vi "getSerializedData.vi"(0 "reference":refnum<class "SegmentedLineEdge.lvclass">, 5 "error in (no error)":errorcluster) -> (14 "reference out":refnum<class "SegmentedLineEdge.lvclass">, 15 "startNode":refnum<class "AbstractNode.lvclass">, 16 "endNode":refnum<class "AbstractNode.lvclass">, 17 "xmlOut":string, 19 "error out":errorcluster)   [LabVIEW 2020, in "SegmentedLineEdge.lvclass"]
doc: "getSerializedData"
uses:
  <resource>/Framework/Providers/Open_GDS/UML/SegmentedLineEdge_class/SegmentedLineEdge.lvclass
  C:/Program Files (x86)/National Instruments/LabVIEW 2020/resource/Framework/Providers/Open_GDS/UML/AbstractEdge_class/AbstractEdge.lvclass
  <resource>/Framework/Providers/Open_GDS/UML/AbstractNode_class/AbstractNode.lvclass
  <resource>/Framework/Providers/Open_GDS/UML/General/Point/Point Point2D.ctl
  <resource>/Framework/Providers/Open_GDS/UML/ArrowHead_class/ArrowHead.lvclass
  <resource>/Framework/Providers/Open_GDS/UML/LineStyle_class/LineStyle.lvclass
  <resource>/Framework/Providers/Open_GDS/UML/AbstractEdge_class/AbstractEdge.lvclass
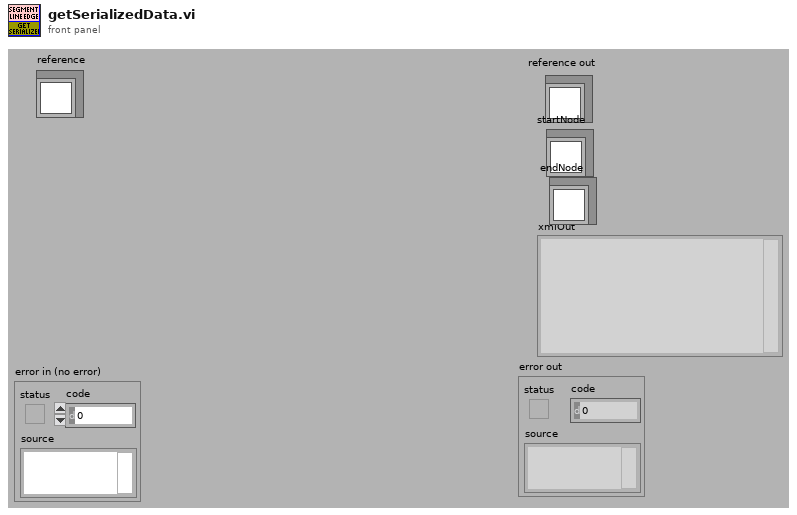
[diagram p1: front panel]
types:
  T1 = typedef "Point Point2D.ctl" = cluster{"x":dbl, "y":dbl}
  T2 = cluster{"Base class":cluster{"Base class":cluster{"start":refnum<k1>, "end":refnum<k1>}}, "lineStyle":refnum<k1>, "startArrowHead":refnum<k1>, "endArrowHead":refnum<k1>, "startLabel":string, "midLabel":string, "endLabel":string, "MidLabelOffset":T1, "SplitWire":bool}
  T3 = typedef "SegmentedLineEdge.lvclass/ObjectAttributes.ctl" = cluster{"lineStyle":refnum<class "LineStyle.lvclass">, "startArrowHead":refnum<class "ArrowHead.lvclass">, "endArrowHead":refnum<class "ArrowHead.lvclass">, "startLabel":string, "midLabel":string, "endLabel":string, "MidLabelOffset":T1, "SplitWire":bool}
  T4 = typedef "AbstractEdge.lvclass/ObjectAttributes.ctl" = cluster{"start":refnum<class "AbstractNode.lvclass">, "end":refnum<class "AbstractNode.lvclass">}
  T5 = cluster{"Base class":cluster{"Base class":cluster{"Base class":cluster{"start":refnum<k1>, "end":refnum<k1>}}, "lineStyle":refnum<k1>, "startArrowHead":refnum<k1>, "endArrowHead":refnum<k1>, "startLabel":string, "midLabel":string, "endLabel":string, "MidLabelOffset":T1, "SplitWire":bool}, "Type(String)":string, "Object name":string, "Object name":string}
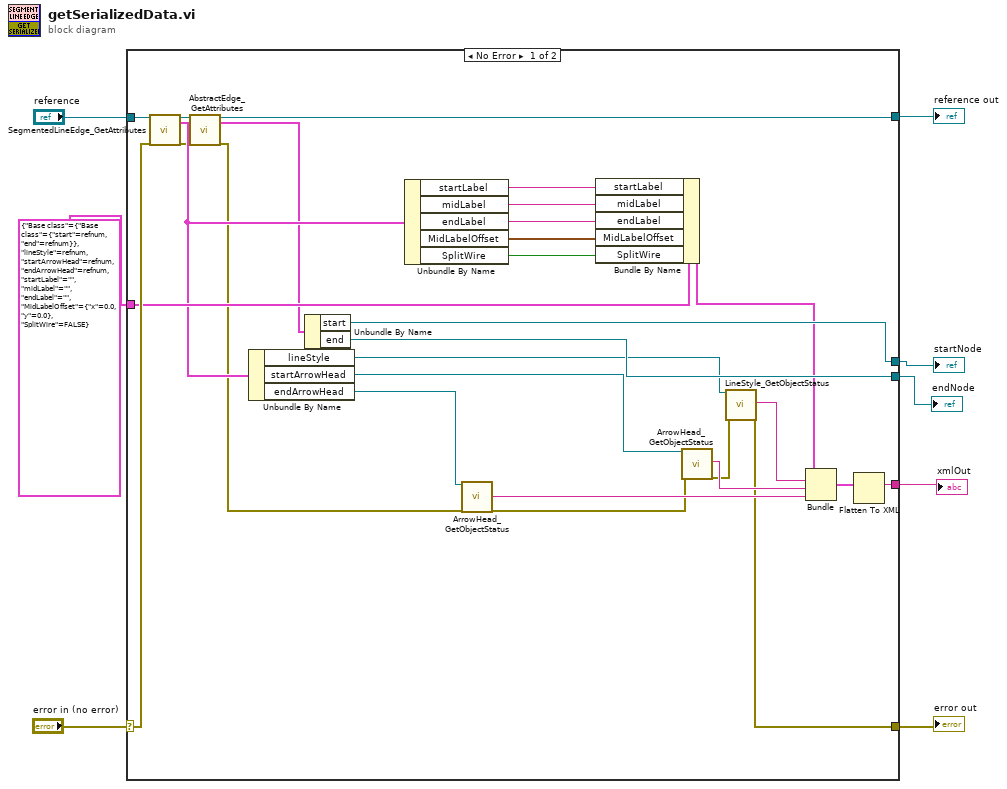
[diagram p0: block diagram]
diagram:
  n1 = case shown="No Error" "error in (no error)" {
    selector: "error in (no error)" -> [w36 w37]
    tunnel: "reference" -> [w35 w38]
    tunnel: [w9 w37] -> w6
    tunnel: [w16 w38] -> w5
    tunnel: [w33 _] -> w4
    tunnel: [w32 _] -> w3
    tunnel: [w31 _] -> w2
    tunnel: T2 {"Base class"={"Base class"={"start"=refnum, "end"=refnum}}, "lineStyle"=refnum, "startArrowHead"=refnum, "endArrowHead"=refnum, "startLabel"="", "midLabel"="", "endLabel"="", "MidLabelOffset"={"x"=0.0, "y"=0.0}, "SplitWire"=FALSE} ("Base class") -> [w22 _]
    frame No Error {
      n2 = call <resource>:"SegmentedLineEdge_GetAttributes.vi"("reference in"=w35, "error in (no error)"=w36) -> ("reference out"=w19:refnum<class "SegmentedLineEdge.lvclass">, "Data"=w20:T3, "error out"=w18:errorcluster)  [unwired: 1 in, 14 out]
      n3 = call <resource>:"AbstractEdge_GetAttributes.vi"("reference in"=w19, "error in (no error)"=w18) -> ("reference out"=w16:refnum<class "SegmentedLineEdge.lvclass">, "Data"=w15:T4, "error out"=w17:errorcluster)  [unwired: 14 in, 1 out]
      n4 = Unbundle By Name(w20) -> ("lineStyle"=w30:refnum<class "LineStyle.lvclass">, "startArrowHead"=w29:refnum<class "ArrowHead.lvclass">, "endArrowHead"=w28:refnum<class "ArrowHead.lvclass">)
      n5 = Unbundle By Name(w15) -> ("start"=w32:refnum<class "AbstractNode.lvclass">, "end"=w31:refnum<class "AbstractNode.lvclass">)
      n6 = Unbundle By Name(w20) -> ("startLabel"=w27:string, "midLabel"=w26:string, "endLabel"=w25:string, "MidLabelOffset"=w24:T1, "SplitWire"=w23:bool)
      n7 = call <resource>:"ArrowHead_GetObjectStatus.vi"("reference in"=w28, "error in (no error)"=w17) -> ("Object name"=w12:string, "error out"=w11:errorcluster)  [unwired: 1 in, 15 out]
      n8 = Bundle By Name(cluster=w22, "startLabel"=w27, "midLabel"=w26, "endLabel"=w25, "MidLabelOffset"=w24, "SplitWire"=w23) -> (w21:T2)
      n9 = call <resource>:"ArrowHead_GetObjectStatus.vi"("reference in"=w29, "error in (no error)"=w11) -> ("Object name"=w13:string, "error out"=w10:errorcluster)  [unwired: 1 in, 15 out]
      n10 = call <resource>:"LineStyle_GetObjectStatus.vi"("reference"=w30, "error in (no error)"=w10) -> ("Type(String)"=w14:string, "error out"=w9:errorcluster)  [unwired: 15 in, 1 out]
      n11 = Bundle("Base class"=w21, "Type(String)"=w14, "Object name"=w13, "Object name"=w12) -> (w34:T5)  [unwired: 1 out]
      n12 = Flatten To XML(6:w34) -> (2:w33:string)
    }
    frame Error {
    }
  }
  "reference out" <- w5
  "error out" <- w6
  "startNode" <- w3
  "endNode" <- w2
  "xmlOut" <- w4
